vi "Read Type Definition.vi"(8 "error in":errorcluster, 11 "Cluster in":refnum<class "Cluster.lvclass">) -> (0 "error out":errorcluster, 2 "Type Definition":path, 3 "Cluster out":refnum<class "Cluster.lvclass">)   [LabVIEW 2026, in "Cluster.lvclass"]
doc: "Data accessor."
uses:
  Cluster.lvclass
  Cluster.lvclass/Cluster.ctl
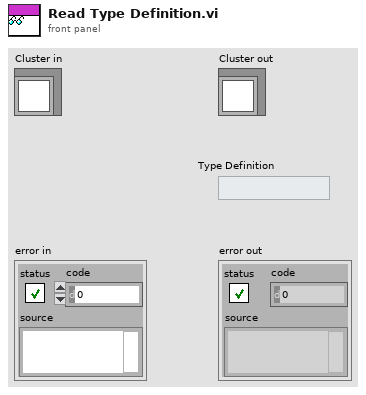
[diagram p1: front panel]
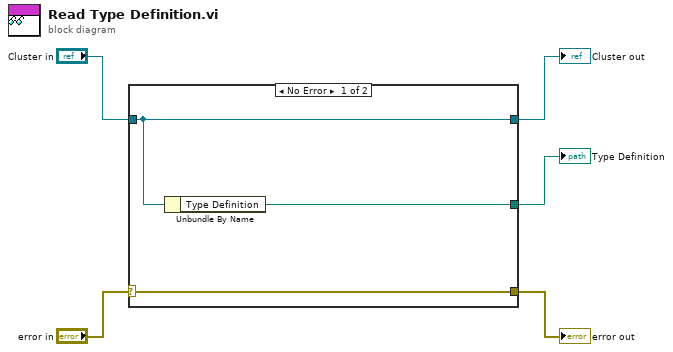
[diagram p0: block diagram]
diagram:
  n1 = case shown="No Error" "error in" {
    selector: "error in" -> [w8 w10]
    tunnel: [w8 w10] -> w4
    tunnel: [w7 w9] -> w2
    tunnel: "Cluster in" -> [w7 w9]
    tunnel: [w6 _] -> w1
    frame No Error {
      n2 = Unbundle By Name(w7) -> ("Type Definition"=w6:path)
    }
    frame Error {
      # "Pass error without further action."
    }
  }
  "error out" <- w4
  "Cluster out" <- w2
  "Type Definition" <- w1
